vi "F2_Read_Array.vi"(10 "Format":string, 11 "File Path":path) -> (1 "error out":errorcluster, 2 "Text":string, 3 "Data":dbl[][](array[numeric]))   [LabVIEW 2018]
doc: "Use this template to build a VI to use as a subVI."
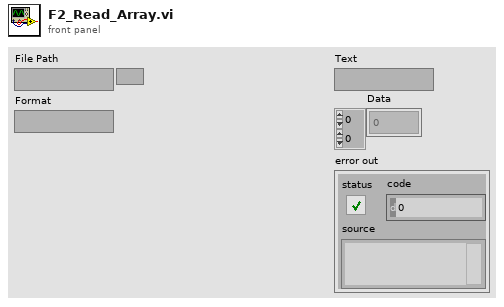
[diagram p1: front panel]
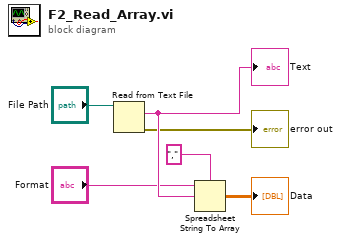
[diagram p0: block diagram]
diagram:
  n1 = Read from Text File(file (use dialog)="File Path") -> (text=w5:string, error out=→"error out":errorcluster)  [unwired: 3 in, 2 out]
  "Text" <- w5
  n2 = Spreadsheet String To Array(delimiter (Tab)=",", format string="Format", spreadsheet string=w5) -> (array=→"Data":dbl[][])  [unwired: 1 in]
